vi "Bridge_Dispatch.vi"(8 "error in (no error)":errorcluster={"status"=FALSE, "code"=0, "source"="\"\""}, 10 "adapter registry":string, 11 "Authorized request":string) -> (0 "error out":errorcluster={"status"=FALSE, "code"=0, "source"="\"\""}, 2 "status ok":bool, 3 "Dispatch ticket":string)   [LabVIEW 2026]
doc: "INTENT: Route validated typed command. LOGIC: Translate logical action to physical adapter protocol, send command with bounded queue depth."
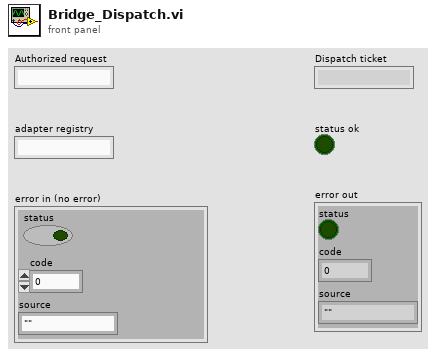
[diagram p1: front panel]
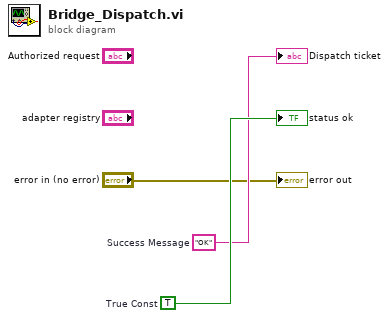
[diagram p0: block diagram]
diagram:
  w3 = TRUE  # True Const
  w2 = "OK"  # Success Message
  "Dispatch ticket" <- w2
  "status ok" <- w3
  "error out" <- "error in (no error)"
